vi "INL-DNL-Status.vi"() -> ()   [LabVIEW 2026, in "Core.lvlib"]
uses:
  Core.lvlib
panel:
  out "INL Plot":dbl[](graph)
  out "INL":dbl
  out "Codes":u32
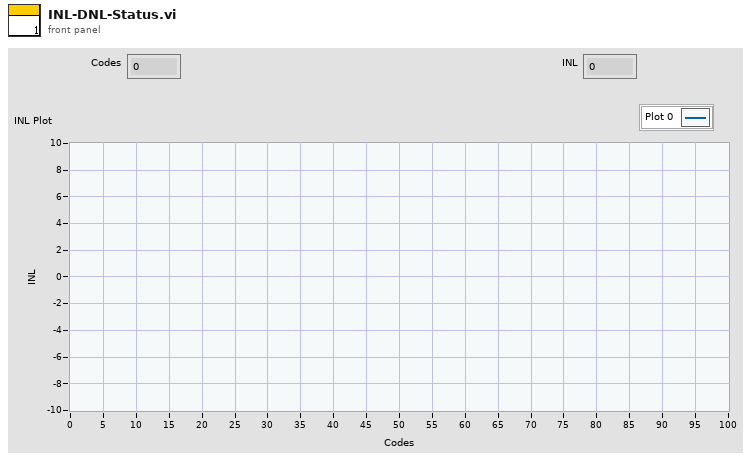
[diagram p1: front panel]
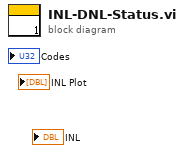
[diagram p0: block diagram]
diagram:
